vi "tab control refresh.vi"(6 "c header file path":path, 8 "error in":errorcluster, 9 "output file string":string, 10 "input file string":string, 11 "VI reference":refnum<vi>) -> (0 "error out":errorcluster)   [LabVIEW 2014, in "Shared Memory editor node.lvclass"]
doc: "***TODO***\n\n<B>Input Parameters</B>\n\n<B>error in</B> describes error conditions that occur before this node runs. This input provides standard error in functionality.\n\n<B>write directory</B> ***TODO***write directory\n\n<B>read directory</B> ***TODO***read directory\n\n<B>VI reference</B> ***TODO***VI reference\n\n<B>Output Parameters</B>\n\n<B>error out</B> contains error information. This output provides standard error out functionality."
uses:
  Shared Memory editor node.lvclass
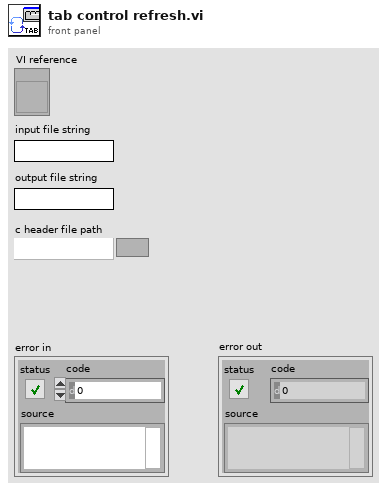
[diagram p1: front panel]
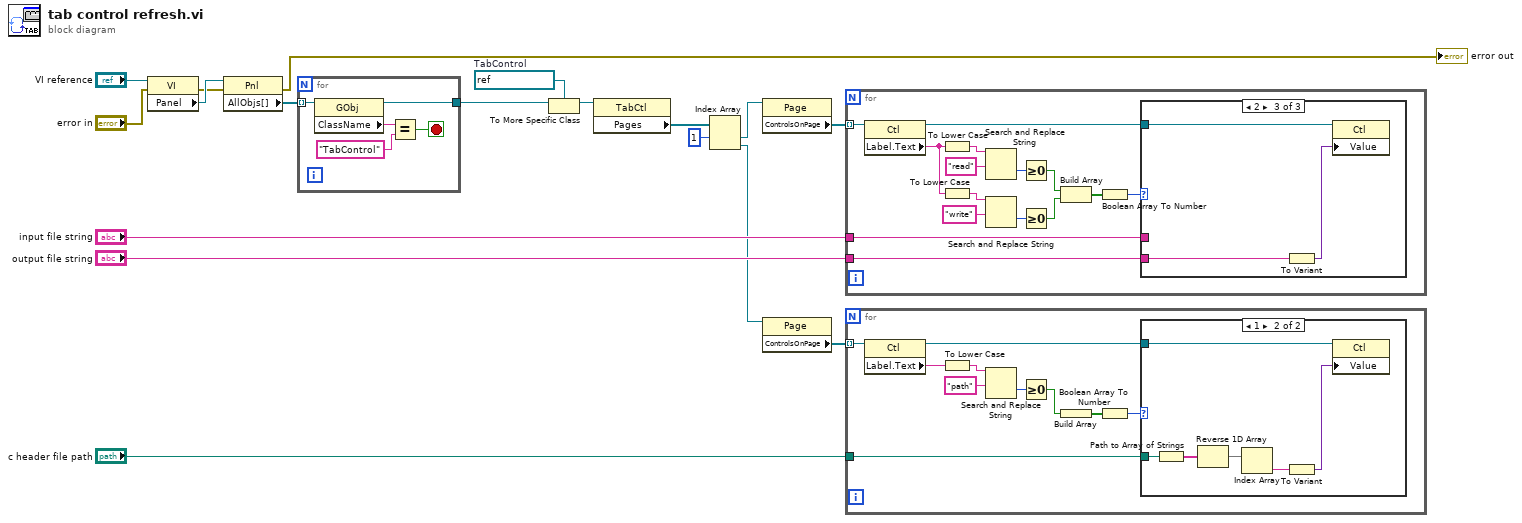
[diagram p0: block diagram]
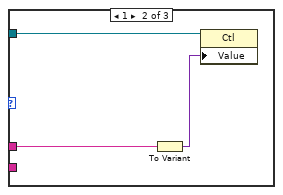
[diagram p4: hidden frame]
diagram:
  w13 = refnum<vi> refnum  # TabControl
  n1 = property class="VI"(reference="VI reference", error in="error in") -> (error out=w9:errorcluster, "Panel"=w11:refnum<vi>)  [unwired: 1 out]
  n2 = property class="Pnl"(reference=w11, error in=w9) -> (error out=→"error out":errorcluster, "AllObjs[]"=w10:refnum<vi>[])  [unwired: 1 out]
  n3 = for {
    tunnel: w10 -> [w23] mode=indexing
    tunnel: [w22] -> w12
    stop <- w19 stop-if-true
    n4 = property class="GObj"(reference=w23) -> (reference out=w22:refnum<vi>, "ClassName"=w20:string)  [unwired: 1 in, 1 out]
    n5 = Equal?(x=w20, y="TabControl") -> (x = y?=w19:bool)
  }
  n6 = To More Specific Class(target class=w13, reference=w12) -> (specific class reference=w14:refnum<vi>)  [unwired: 1 in, 1 out]
  n7 = property class="TabCtl"(reference=w14) -> ("Pages"=w15:refnum<vi>[])  [unwired: 1 in, 2 out]
  n8 = Index Array(array=w15, index #1=1 ("index")) -> (element #1=w17:refnum<vi>, element #2=w1:refnum<vi>)  [unwired: 1 in]
  n9 = property class="Page"(reference=w17) -> ("ControlsOnPage"=w18:refnum<vi>[])  [unwired: 1 in, 2 out]
  n10 = property class="Page"(reference=w1) -> ("ControlsOnPage"=w3:refnum<vi>[])  [unwired: 1 in, 2 out]
  n11 = for {
    tunnel: w18 -> [w38] mode=indexing
    tunnel: "input file string" -> [w25]
    tunnel: "output file string" -> [w24]
    n12 = property class="Ctl"(reference=w38) -> (reference out=w37:refnum<vi>, "Label.Text"=w32:string)  [unwired: 1 in, 1 out]
    n13 = To Lower Case(string=w32) -> (all lower case string=w36:string)
    n14 = To Lower Case(string=w32) -> (all lower case string=w33:string)
    n15 = Search and Replace String(input string=w36, search string="read") -> (offset past replacement=w31:i32)  [unwired: 6 in, 3 out]
    n16 = Search and Replace String(input string=w33, search string="write") -> (offset past replacement=w30:i32)  [unwired: 6 in, 3 out]
    n17 = Greater Or Equal To 0?(x=w31) -> (x >= 0?=w29:bool)
    n18 = Greater Or Equal To 0?(x=w30) -> (x >= 0?=w28:bool)
    n19 = Build Array(w29, w28) -> (w27:bool[])
    n20 = Boolean Array To Number(Boolean array=w27) -> (number=w26:u32)
    n21 = case shown="2" w26 {
      tunnel: w37 -> [_ w41 w44]
      tunnel: w25 -> [_ w39 _]
      tunnel: w24 -> [_ _ w42]
      frame Default {
      }
      frame 1 {
        n22 = To Variant(anything=w39) -> (Variant=w40:variant)
        n23 = property class="Ctl"(reference=w41, "Value"=w40) -> ()  [unwired: 1 in, 2 out]
      }
      frame 2 {
        n24 = To Variant(anything=w42) -> (Variant=w43:variant)
        n25 = property class="Ctl"(reference=w44, "Value"=w43) -> ()  [unwired: 1 in, 2 out]
      }
    }
  }
  n26 = for {
    tunnel: w3 -> [w54] mode=indexing
    tunnel: "c header file path" -> [w45]
    n27 = property class="Ctl"(reference=w54) -> (reference out=w53:refnum<vi>, "Label.Text"=w50:string)  [unwired: 1 in, 1 out]
    n28 = To Lower Case(string=w50) -> (all lower case string=w52:string)
    n29 = Search and Replace String(input string=w52, search string="path") -> (offset past replacement=w49:i32)  [unwired: 6 in, 3 out]
    n30 = Greater Or Equal To 0?(x=w49) -> (x >= 0?=w48:bool)
    n31 = Build Array(w48) -> (w47:bool[])
    n32 = Boolean Array To Number(Boolean array=w47) -> (number=w46:u32)
    n33 = case shown="1" w46 {
      tunnel: w53 -> [_ w60]
      tunnel: w45 -> [_ w58]
      frame Default {
      }
      frame 1 {
        n34 = Path to Array of Strings(0:w58) -> (2:w57:string[])  [unwired: 1 out]
        n35 = Reverse 1D Array(array=w57) -> (reversed array=w56:string[])
        n36 = Index Array(array=w56) -> (element=w55:string)  [unwired: 1 in]
        n37 = To Variant(anything=w55) -> (Variant=w59:variant)
        n38 = property class="Ctl"(reference=w60, "Value"=w59) -> ()  [unwired: 1 in, 2 out]
      }
    }
  }
